vi "Find All IO Variables.vi"(8 "error in":errorcluster, 10 "Path":path) -> (0 "error out":errorcluster, 2 "Tags":T1[](array[typedef]))   [LabVIEW 2015, in "Scan Engine editor node.lvclass"]
uses:
  Scan Engine editor node.lvclass
  configuration/Line.ctl
  <vilib>/NI/Tag Bus Module Framework/channel/TBM channel.lvclass
  <vilib>/NI/Tag Bus Module Framework/channel/channel classification.ctl
  <vilib>/NI/Tag Bus/tag/Data Type.ctl
  <vilib>/Utility/VariantDataType/VariantType.lvlib
  <vilib>/NI/Tag Bus/tag/tag descriptor.lvclass
  configuration/Scan Engine configuration.lvclass
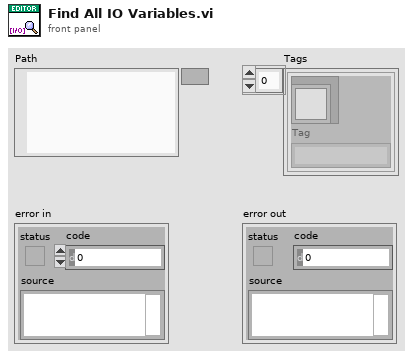
[diagram p1: front panel]
types:
  T1 = typedef "Scan Engine configuration.lvclass/Line.ctl" = cluster{"channel":refnum<class "TBM channel.lvclass">, "Tag":string}
  T2 = typedef "TBM channel.lvclass/channel classification.ctl" = enum16{"input data", "output data", "processing parameter", "processing result"}
  T3 = typedef "tag bus.lvlib/tag descriptor.lvclass/Data Type.ctl" = enum16{"Double", "Single", "I64", "I32", "I16", "I8", "U64", "U32", "U16", "U8", "Boolean", "String", "Array of Double", "Array of Single", "Array of I64", "Array of I32", "Array of I16", "Array of I8", "Array of U64", "Array of U32", "Array of U16", "Array of U8", "Array of Boolean", "Array of String"}
  T4 = enum16{"Single-Process", "Network-Published", "Time-Triggered", "Industrial"}
  T5 = typedef "VariantType.lvlib/Type.ctl" = enum8{"Invalid Type", "Void", "I8", "I16", "I32", "I64", "U8", "U16", "U32", "U64", "Single Float", "Double Float", "Extended Float", "Single Complex", "Double Complex", "Extended Complex", "Enum U8", "Enum U16", "Enum U32", "Enum U64", "Single Float With Unit", "Double Float With Unit", "Extended Float With Unit", "Single Complex with Unit", "Double Complex with Unit", "Extended Complex with Unit", "Boolean", "String", "Path", "Picture", "Tag", "Array", "Cluster", "Variant", "LV Variant", "Waveform", "Timestamp", "Digital Waveform", "Digital Data", "ExpressData", "Refnum", "External Data", "VI", "Poly VI", "LabVIEW Class Instance", "Fixed Point"}
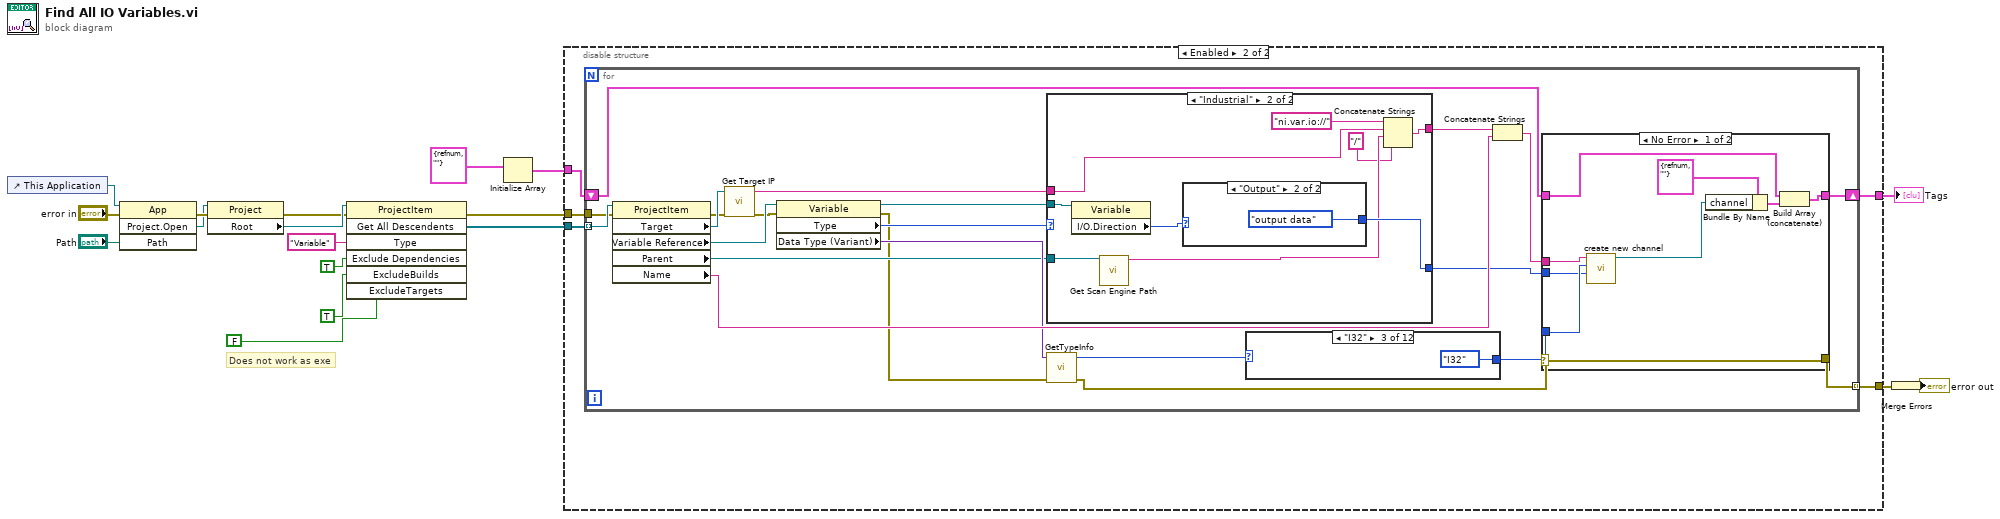
[diagram p0: block diagram]
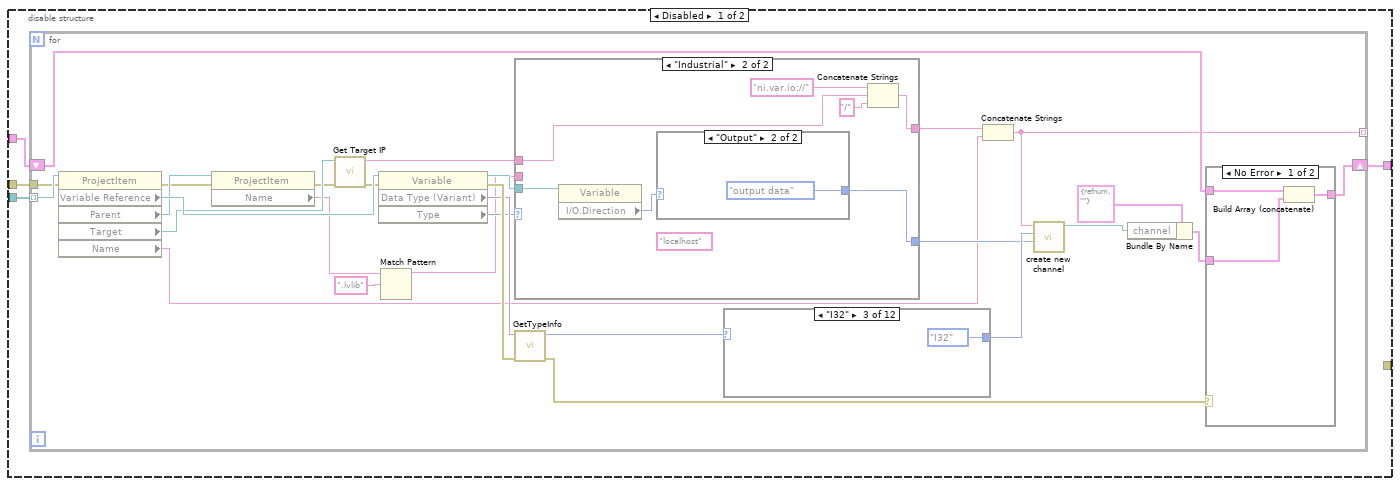
[diagram p2: hidden frame]
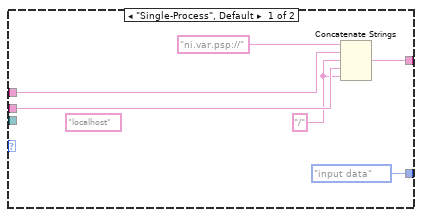
[diagram p3: hidden frame]
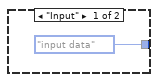
[diagram p4: hidden frame]
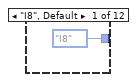
[diagram p6: hidden frame]
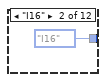
[diagram p7: hidden frame]
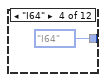
[diagram p8: hidden frame]
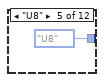
[diagram p9: hidden frame]
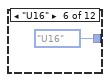
[diagram p10: hidden frame]
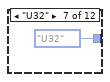
[diagram p11: hidden frame]
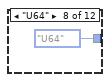
[diagram p12: hidden frame]
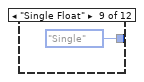
[diagram p13: hidden frame]
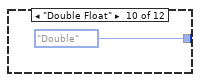
[diagram p14: hidden frame]
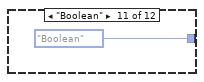
[diagram p15: hidden frame]
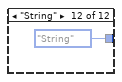
[diagram p16: hidden frame]
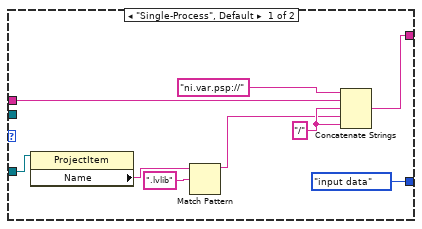
[diagram p17: hidden frame]
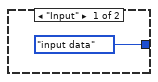
[diagram p18: hidden frame]
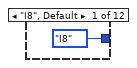
[diagram p20: hidden frame]
diagram:
  # "Does not work as exe"
  n1 = control-ref of="This Application"() -> (w14:refnum<vi>)
  n2 = invoke class="App" method="Project.Open"(reference=w14, error in="error in", "Path"="Path") -> (error out=w16:errorcluster, "Project:Open"=w15:refnum<vi>)  [unwired: 1 in, 2 out]
  n3 = property class="Project"(reference=w15, error in=w16) -> (error out=w3:errorcluster, "Root"=w5:refnum<vi>)  [unwired: 1 out]
  n4 = invoke class="ProjectItem" method="Get All Descendents"(reference=w5, error in=w3, "Type"="Variable", "Exclude Dependencies"=TRUE ("ExcludeDependencies"), "ExcludeBuilds"=TRUE, "ExcludeTargets"=FALSE) -> (error out=w4:errorcluster, "All Descendents"=w12:refnum<vi>[])  [unwired: 1 in, 5 out]
  n5 = Initialize Array(T1 {"channel"=refnum, "Tag"=""} ("Line")) -> (w7:T1[])  [unwired: 1 in]
  n6 = disable-structure shown="Enabled" {
    disable-tunnel: w12 -> [w22 w86]
    disable-tunnel: w7 -> [w21 w85]
    disable-tunnel: [w20 w84] -> w6
    disable-tunnel: w4 -> [w19 w83]
    disable-tunnel: [_ w82] -> w2
    frame Disabled {
      n7 = for {
        tunnel: w22 -> [w50] mode=indexing
        shift-right: [w41] -> w20
        shift-left: w21 -> [w40]
        tunnel: [w36] -> _ mode=indexing
        tunnel: w19 -> [w30]
        n8 = property class="ProjectItem"(reference=w50, error in=w30) -> (error out=w29:errorcluster, "Variable Reference"=w39:refnum<vi>, "Parent"=w33:refnum<vi>, "Target"=w35:refnum<vi>, "Name"=w23:string)  [unwired: 1 out]
        n9 = property class="ProjectItem"(reference=w33, error in=w29) -> (error out=w28:errorcluster, "Name"=w32:string)  [unwired: 1 out]
        n10 = call "Get Target IP.vi"("error in (no error)"=w28, "TargetItem in"=w35) -> ("error out"=w27:errorcluster, "string"=w34:string)  [unwired: 8 in]
        n11 = property class="Variable"(reference=w39, error in=w27) -> (reference out=w26:refnum<vi>, error out=w49:errorcluster, "Data Type (Variant)"=w46:variant, "Type"=w38:T4)
        n12 = Match Pattern(string=w32, regular expression=".lvlib") -> (before substring=w25:string)  [unwired: 1 in, 3 out]
        n13 = case shown="\"Industrial\"" w38 {
          tunnel: [w55 w61] -> w37
          tunnel: w34 -> [w54 w60]
          tunnel: w25 -> [w53 _]
          tunnel: w26 -> [_ w59]
          tunnel: [channel_classification."input data" ("channel classification") w57] -> w24
          frame "Single-Process", Default {
            (unwired) "localhost" ("string")
            w52 = "/" ("string")
            n14 = Concatenate Strings("ni.var.psp://", w54, w52, w53, w52) -> (w55:string)
          }
          frame "Industrial" {
            (unwired) "localhost" ("string")
            n15 = property class="Variable"(reference=w59) -> ("I/O.Direction"=w58:enum8{"Input", "Output"})  [unwired: 1 in, 2 out]
            n16 = case shown="\"Output\"" w58 {
              tunnel: [channel_classification."input data" ("channel classification") channel_classification."output data" ("channel classification")] -> w57
              frame "Input" {
              }
              frame "Output" {
              }
            }
            n17 = Concatenate Strings("ni.var.io://", w60, "/" ("string")) -> (w61:string)
          }
        }
        n18 = call <vilib>:"GetTypeInfo.vi"("error in (no error)"=w49, "Variant"=w46) -> ("error out"=w43:errorcluster, "Type Enum"=w48:T5)  [unwired: 5 in, 3 out]
        n19 = case shown="\"I32\"" w48 {
          tunnel: [Data_Type."I8" ("data type") Data_Type."I16" ("data type") Data_Type."I32" ("data type") Data_Type."I64" ("data type") Data_Type."U8" ("data type") Data_Type."U16" ("data type") Data_Type."U32" ("data type") Data_Type."U64" ("data type") Data_Type."Single" ("data type") Data_Type."Double" ("data type") Data_Type."Boolean" ("data type") Data_Type."String" ("data type")] -> w45
          frame "I8", Default {
          }
          frame "I16" {
          }
          frame "I32" {
          }
          frame "I64" {
          }
          frame "U8" {
          }
          frame "U16" {
          }
          frame "U32" {
          }
          frame "U64" {
          }
          frame "Single Float" {
          }
          frame "Double Float" {
          }
          frame "Boolean" {
          }
          frame "String" {
          }
        }
        n20 = Concatenate Strings(w37, w23) -> (w36:string)
        n21 = call <vilib>:"create new channel.vi"("channel classification"=w24, "data type"=w45, "channel name"=w36) -> ("channel"=w44:refnum<class "TBM channel.lvclass">)  [unwired: 8 in]
        n22 = Bundle By Name(cluster=T1 {"channel"=refnum, "Tag"=""} ("Line"), "channel"=w44) -> (w47:T1)
        n23 = case shown="No Error" w43 {
          tunnel: w40 -> [w68 w69]
          tunnel: [w67 w69] -> w41
          tunnel: w47 -> [w66 _]
          frame No Error {
            n24 = Build Array (concatenate)(w68, w66) -> (w67:T1[])
          }
          frame Error {
          }
        }
      }
    }
    frame Enabled {
      n25 = for {
        tunnel: w86 -> [w108] mode=indexing
        shift-right: [w105] -> w84
        shift-left: w85 -> [w104]
        tunnel: w83 -> [w100]
        tunnel: [w93] -> w82 mode=indexing
        n26 = property class="ProjectItem"(reference=w108, error in=w100) -> (error out=w90:errorcluster, "Target"=w91:refnum<vi>, "Variable Reference"=w92:refnum<vi>, "Parent"=w89:refnum<vi>, "Name"=w98:string)  [unwired: 1 out]
        n27 = call "Get Target IP.vi"("error in (no error)"=w90, "TargetItem in"=w91) -> ("error out"=w88:errorcluster, "string"=w101:string)  [unwired: 8 in]
        n28 = property class="Variable"(reference=w92, error in=w88) -> (reference out=w99:refnum<vi>, error out=w87:errorcluster, "Type"=w103:T4, "Data Type (Variant)"=w94:variant)
        n29 = case shown="\"Industrial\"" w103 {
          tunnel: [w116 w125] -> w102
          tunnel: w101 -> [w115 w124]
          tunnel: w99 -> [_ w123]
          tunnel: [channel_classification."input data" ("channel classification") w121] -> w95
          tunnel: w89 -> [w110 w120]
          frame "Single-Process", Default {
            w114 = "/" ("string")
            n30 = property class="ProjectItem"(reference=w110) -> ("Name"=w111:string)  [unwired: 1 in, 2 out]
            n31 = Match Pattern(string=w111, regular expression=".lvlib") -> (before substring=w109:string)  [unwired: 1 in, 3 out]
            n32 = Concatenate Strings("ni.var.psp://", w115, w114, w109, w114) -> (w116:string)
          }
          frame "Industrial" {
            n33 = property class="Variable"(reference=w123) -> ("I/O.Direction"=w122:enum8{"Input", "Output"})  [unwired: 1 in, 2 out]
            n34 = call "Get Scan Engine Path.vi"("ProjectItem in"=w120) -> ("Path"=w119:string)  [unwired: 10 in]
            n35 = case shown="\"Output\"" w122 {
              tunnel: [channel_classification."input data" ("channel classification") channel_classification."output data" ("channel classification")] -> w121
              frame "Input" {
              }
              frame "Output" {
              }
            }
            n36 = Concatenate Strings("ni.var.io://", w124, w119, "/" ("string")) -> (w125:string)
          }
        }
        n37 = call <vilib>:"GetTypeInfo.vi"("error in (no error)"=w87, "Variant"=w94) -> ("error out"=w106:errorcluster, "Type Enum"=w107:T5)  [unwired: 5 in, 3 out]
        n38 = case shown="\"I32\"" w107 {
          tunnel: [Data_Type."I8" ("data type") Data_Type."I16" ("data type") Data_Type."I32" ("data type") Data_Type."I64" ("data type") Data_Type."U8" ("data type") Data_Type."U16" ("data type") Data_Type."U32" ("data type") Data_Type."U64" ("data type") Data_Type."Single" ("data type") Data_Type."Double" ("data type") Data_Type."Boolean" ("data type") Data_Type."String" ("data type")] -> w96
          frame "I8", Default {
          }
          frame "I16" {
          }
          frame "I32" {
          }
          frame "I64" {
          }
          frame "U8" {
          }
          frame "U16" {
          }
          frame "U32" {
          }
          frame "U64" {
          }
          frame "Single Float" {
          }
          frame "Double Float" {
          }
          frame "Boolean" {
          }
          frame "String" {
          }
        }
        n39 = Concatenate Strings(w102, w98) -> (w97:string)
        n40 = case shown="No Error" w106 {
          selector: w106 -> [w129 w138]
          tunnel: w104 -> [w137 w139]
          tunnel: [w136 w139] -> w105
          tunnel: w97 -> [w132 _]
          tunnel: w96 -> [w131 _]
          tunnel: w95 -> [w130 _]
          tunnel: [w129 w138] -> w93
          frame No Error {
            n41 = call <vilib>:"create new channel.vi"("channel classification"=w130, "data type"=w131, "channel name"=w132) -> ("channel"=w134:refnum<class "TBM channel.lvclass">)  [unwired: 8 in]
            n42 = Bundle By Name(cluster=T1 {"channel"=refnum, "Tag"=""} ("Line"), "channel"=w134) -> (w133:T1)
            n43 = Build Array (concatenate)(w137, w133) -> (w136:T1[])
          }
          frame Error {
          }
        }
      }
    }
  }
  "Tags" <- w6
  n44 = Merge Errors(w2) -> (→"error out":errorcluster)
